vi "Write Variant OPC.vi"(8 "error in (no error)":errorcluster, 10 "data":variant, 11 "URL":string) -> (0 "error out":errorcluster, 3 "Desc":string)   [LabVIEW 2012]
uses:
  write_Array.vi
  Globals/Global.vi
  write_String.vi
  write_bool.vi
  write_Num.vi
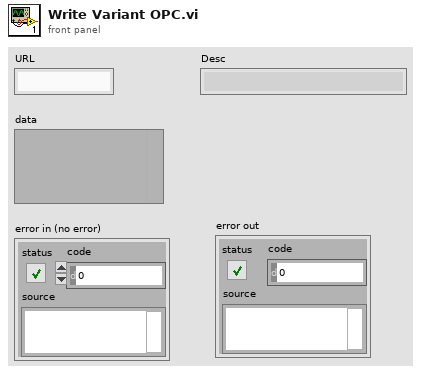
[diagram p1: front panel]
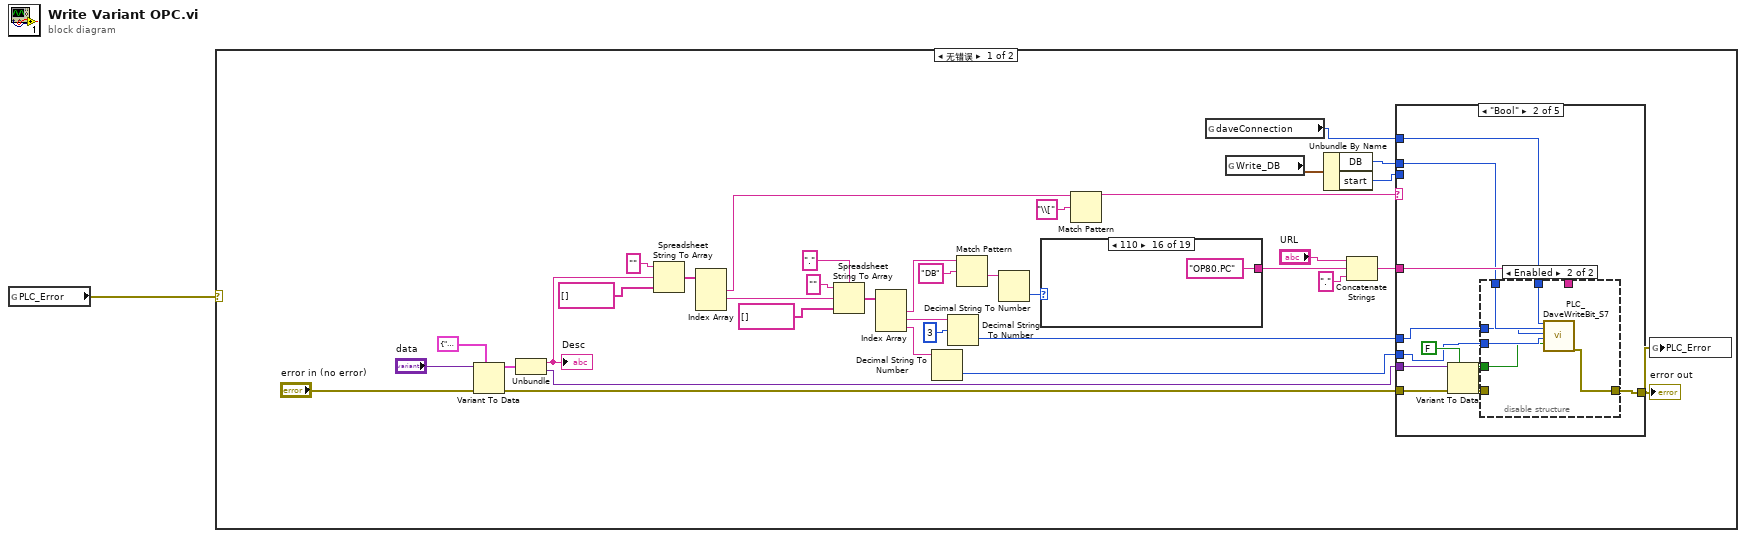
[diagram p0: block diagram]
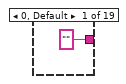
[diagram p2: hidden frame]
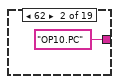
[diagram p3: hidden frame]
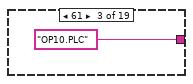
[diagram p4: hidden frame]
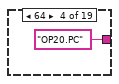
[diagram p5: hidden frame]
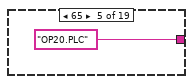
[diagram p6: hidden frame]
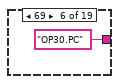
[diagram p7: hidden frame]
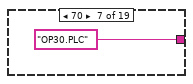
[diagram p8: hidden frame]
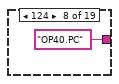
[diagram p9: hidden frame]
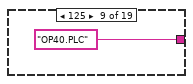
[diagram p10: hidden frame]
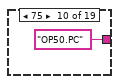
[diagram p11: hidden frame]
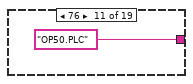
[diagram p12: hidden frame]
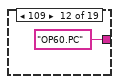
[diagram p13: hidden frame]
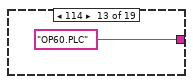
[diagram p14: hidden frame]
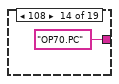
[diagram p15: hidden frame]
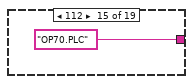
[diagram p16: hidden frame]
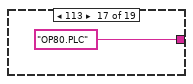
[diagram p17: hidden frame]
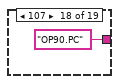
[diagram p18: hidden frame]
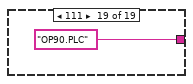
[diagram p19: hidden frame]
diagram:
  n1 = global read "Global.vi" "PLC_Error"() -> (w1:errorcluster)
  n2 = case shown="无错误" w1 {
    frame No Error {
      n3 = Variant To Data(error in="error in (no error)", type=cluster{"Desc":string, "NewVal":variant} {"Desc"="", "NewVal"=variant} ("output cluster"), Variant="data") -> (data=w29:cluster{"Desc":string, "NewVal":variant}, error out=w36:errorcluster)
      n4 = Unbundle(w29) -> ("Desc"=w31:string, "NewVal"=w34:variant)
      "Desc" <- w31
      n5 = Spreadsheet String To Array(format string="", spreadsheet string=w31, array type (2D Dbl)=string[] [] ("Device ID")) -> (array=w33:string[])  [unwired: 1 in]
      n6 = Index Array(array=w33) -> (element #1=w21:string, element #2=w25:string)  [unwired: 3 in, 1 out]
      n7 = Spreadsheet String To Array(delimiter (Tab)=".", format string="", spreadsheet string=w25, array type (2D Dbl)=string[] [] ("Device ID")) -> (array=w23:string[])
      n8 = Index Array(array=w23) -> (element #1=w16:string, element #2=w18:string, element #3=w22:string)  [unwired: 3 in]
      n9 = Decimal String To Number(string=w22) -> (number=w8:i32)  [unwired: 2 in, 1 out]
      n10 = Decimal String To Number(string=w18, offset=3) -> (number=w9:i32)  [unwired: 1 in, 1 out]
      n11 = Match Pattern(string=w16, regular expression="DB") -> (after substring=w14:string)  [unwired: 1 in, 3 out]
      n12 = Decimal String To Number(string=w14) -> (number=w13:i32)  [unwired: 2 in, 1 out]
      n13 = case shown="110" w13 {
        tunnel: ["" ("URL") "OP10.PC" ("URL") "OP10.PLC" ("URL") "OP20.PC" ("URL") "OP20.PLC" ("URL") "OP30.PC" ("URL") "OP30.PLC" ("URL") "OP40.PC" ("URL") "OP40.PLC" ("URL") "OP50.PC" ("URL") "OP50.PLC" ("URL") "OP60.PC" ("URL") "OP60.PLC" ("URL") "OP70.PC" ("URL") "OP70.PLC" ("URL") "OP80.PC" ("URL") "OP80.PLC" ("URL") "OP90.PC" ("URL") "OP90.PLC" ("URL")] -> w11
        frame 0, Default {
        }
        frame 62 {
        }
        frame 61 {
        }
        frame 64 {
        }
        frame 65 {
        }
        frame 69 {
        }
        frame 70 {
        }
        frame 124 {
        }
        frame 125 {
        }
        frame 75 {
        }
        frame 76 {
        }
        frame 109 {
        }
        frame 114 {
        }
        frame 108 {
        }
        frame 112 {
        }
        frame 110 {
        }
        frame 113 {
        }
        frame 107 {
        }
        frame 111 {
        }
      }
      n14 = Match Pattern(string=w21, regular expression="\\[") -> (before substring=w19:string)  [unwired: 1 in, 3 out]
      n15 = global read "Global.vi" "daveConnection"() -> (w5:i64)
      n16 = global read "Global.vi" "Write_DB"() -> (w4:cluster{"DB":i32, "start":i32, "len":i32})
      n17 = Unbundle By Name(w4) -> ("DB"=w3:i32, "start"=w2:i32)
      n18 = Concatenate Strings("URL", w11, "." ("string")) -> (w10:string)
      n19 = case shown="\"Bool\"" w19 {
        selector: w19 -> [_ _ _ w119 _]
        tunnel: w10 -> [_ w68 w96 w120 w145]
        tunnel: w34 -> [_ w67 w93 w118 w144]
        tunnel: w36 -> [w57 w66 w95 w117 w143]
        tunnel: w9 -> [_ w61 w86 w108 w140]
        tunnel: w8 -> [_ w60 _ _ _]
        tunnel: [w57 w62 w88 w111 w139] -> w6
        tunnel: w5 -> [_ w58 w85 w109 w136]
        tunnel: w3 -> [_ w59 w87 w110 w138]
        tunnel: w2 -> [_ _ _ _ w137]
        frame Default {
        }
        frame "Bool" {
          n20 = Variant To Data(error in=w66, type=FALSE, Variant=w67) -> (data=w64:bool, error out=w63:errorcluster)
          n21 = disable-structure shown="Enabled" {
            disable-tunnel: w68 -> [w77 _]
            disable-tunnel: w64 -> [w76 w79]
            disable-tunnel: w63 -> [w75 _]
            disable-tunnel: [w71 w78] -> w62
            disable-tunnel: w61 -> [w70 w81]
            disable-tunnel: w60 -> [w69 w80]
            disable-tunnel: w59 -> [_ w83]
            disable-tunnel: w58 -> [_ w82]
            frame Disabled {
              n22 = Format Into String(format string="%d_%d", initial string="DB", w70, w69) -> (resulting string=w72:string)  [unwired: 1 in, 1 out]
              n23 = call-poly "OPC Write.vi"("错误输入（无错误）"=w75, "Value"=w76, "Address"=w72, "URL"=w77) -> ("error out"=w71:errorcluster)  [unwired: 6 in, 1 out]
            }
            frame Enabled {
              n24 = call "PLC_DaveWriteBit_S7.vi"("daveConnection IN"=w82, "DB"=w83, "byte"=w81, "bit"=w80, "value"=w79) -> ("error out"=w78:errorcluster)  [unwired: 12 in, 2 out]
            }
          }
        }
        frame "DInt", "Int" {
          n25 = Variant To Data(error in=w95, type=u32 50 ("milliseconds to wait"), Variant=w93) -> (data=w92:u32)  [unwired: 1 out]
          n26 = Format Into String(format string="%d", initial string="DB", w86) -> (resulting string=w89:string)  [unwired: 1 in, 1 out]
          n27 = disable-structure shown="Enabled" {
            disable-tunnel: w96 -> [w100 _]
            disable-tunnel: w92 -> [w99 w104]
            disable-tunnel: w89 -> [w98 _]
            disable-tunnel: [w97 w101] -> w88
            disable-tunnel: w87 -> [_ w107]
            disable-tunnel: w86 -> [_ w106]
            disable-tunnel: w85 -> [_ w105]
            disable-tunnel: u8[] [] ("Buffer") -> [_ w103]
            frame Disabled {
              n28 = call-poly "OPC Write.vi"("Value"=w99, "Address"=w98, "URL"=w100) -> ("error out"=w97:errorcluster)  [unwired: 7 in, 1 out]
            }
            frame Enabled {
              n29 = Type Cast(type=w103, x=w104) -> (*(type *) &x=w102:u8[])
              n30 = call "PLC_DaveWriteBytes_S7.vi"("daveConnectionIN"=w105, "DB"=w107, "start"=w106, "Buffer"=w102) -> ("error out"=w101:errorcluster)  [unwired: 9 in, 2 out]
            }
          }
        }
        frame "String" {
          n31 = Variant To Data(error in=w117, type=w119, Variant=w118) -> (data=w115:string, error out=w116:errorcluster)
          n32 = Format Into String(format string="%d", initial string="DB", w108) -> (resulting string=w112:string)  [unwired: 1 in, 1 out]
          n33 = disable-structure shown="Enabled" {
            disable-tunnel: w120 -> [w125 _]
            disable-tunnel: w116 -> [w124 _]
            disable-tunnel: w115 -> [w123 w132]
            disable-tunnel: w112 -> [w122 _]
            disable-tunnel: [w121 w126] -> w111
            disable-tunnel: w110 -> [_ w135]
            disable-tunnel: w109 -> [_ w134]
            disable-tunnel: w108 -> [_ w133]
            frame Disabled {
              n34 = call-poly "OPC Write.vi"("错误输入（无错误）"=w124, "Value"=w123, "Address"=w122, "URL"=w125) -> ("error out"=w121:errorcluster)  [unwired: 6 in, 1 out]
            }
            frame Enabled {
              n35 = Type Cast(type=u8[] [] ("Buffer"), x=w132) -> (*(type *) &x=w128:u8[])
              n36 = Array Size(array=w128) -> (size(s)=w130:i32)
              n37 = To Unsigned Byte Integer(number=w130) -> (unsigned 8bit integer=w129:u8)
              n38 = Build Array (concatenate)(w129, w128) -> (w127:u8[])
              n39 = call "PLC_DaveWriteBytes_S7.vi"("daveConnectionIN"=w134, "DB"=w135, "start"=w133, "Buffer"=w127) -> ("error out"=w126:errorcluster)  [unwired: 9 in, 2 out]
            }
          }
        }
        frame "Array" {
          n40 = Variant To Data(error in=w143, type=u8[] [] ("Device ID"), Variant=w144) -> (data=w141:u8[])  [unwired: 1 out]
          n41 = disable-structure shown="Enabled" {
            disable-tunnel: w145 -> [w152 _]
            disable-tunnel: w141 -> [w151 w154]
            disable-tunnel: w140 -> [w148 _]
            disable-tunnel: [w146 w153] -> w139
            disable-tunnel: w138 -> [_ w157]
            disable-tunnel: w137 -> [_ w156]
            disable-tunnel: w136 -> [_ w155]
            frame Disabled {
              n42 = Format Into String(format string="%d", initial string="DB", w148) -> (resulting string=w147:string)  [unwired: 1 in, 1 out]
              n43 = call-poly "OPC Write.vi"("Value"=w151, "Address"=w147, "URL"=w152) -> ("error out"=w146:errorcluster)  [unwired: 7 in, 1 out]
            }
            frame Enabled {
              n44 = call "PLC_DaveWriteBytes_S7.vi"("daveConnectionIN"=w155, "DB"=w157, "start"=w156, "Buffer"=w154) -> ("error out"=w153:errorcluster)  [unwired: 9 in, 2 out]
            }
          }
        }
      }
      "error out" <- w6
      n45 = global write "Global.vi" "PLC_Error"(w6) -> ()
    }
    frame Error {
    }
  }
